vi "TypecastControls.vi"(0 "Controls[]":refnum<vi>[](array[refnum]), 5 "Control Name":string, 9 "Control Path In":string[](array[string]), 11 "error In":errorcluster) -> (4 "Sub Controls[]":refnum<vi>[](array[refnum]), 10 "Control Path Out":string[](array[string]), 15 "error out":errorcluster)   [LabVIEW 2016, in "Drona.lvlib" / "GetControlRef.lvlib"]
doc: "Typecasts the control to its respective class and gives the reference of the controls inside it."
uses:
  GetControlRef.lvlib
  Drona.lvlib
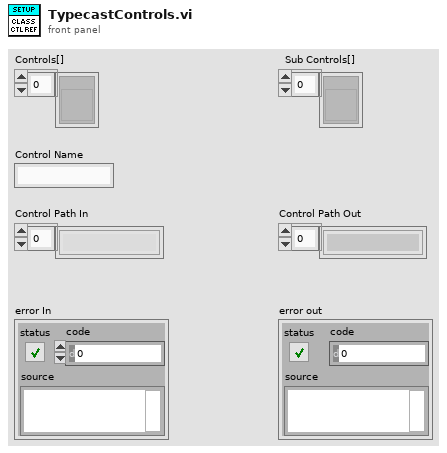
[diagram p1: front panel]
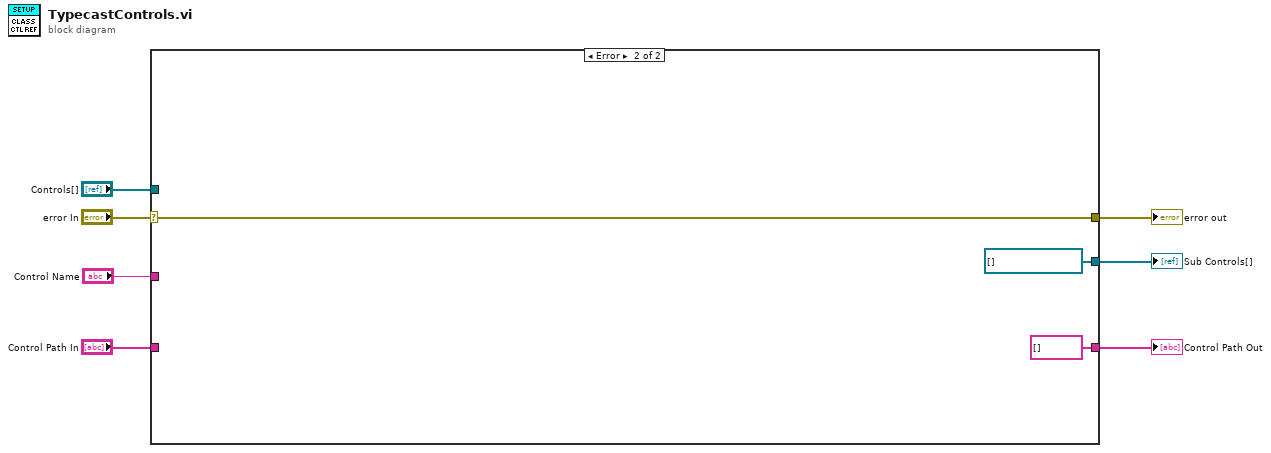
[diagram p0: block diagram]
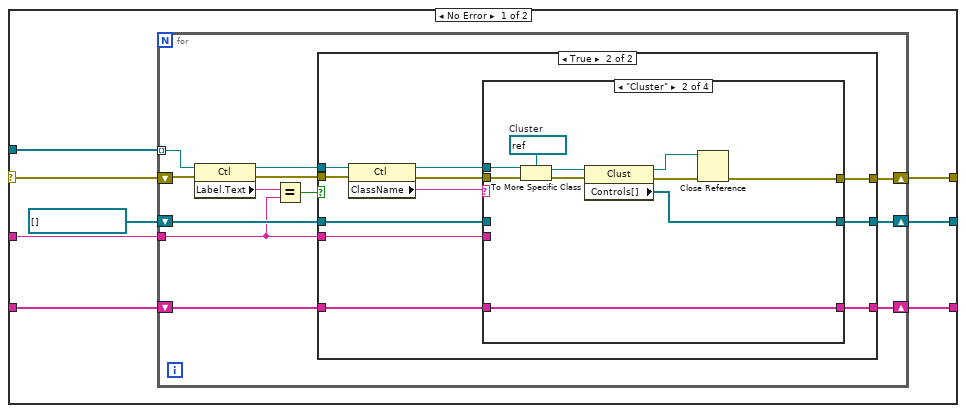
[diagram p2: hidden frame]
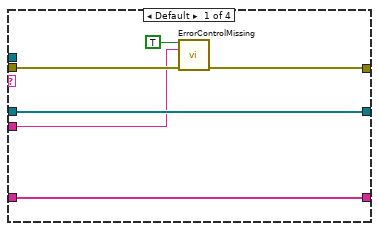
[diagram p4: hidden frame]
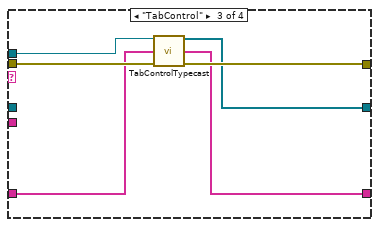
[diagram p5: hidden frame]
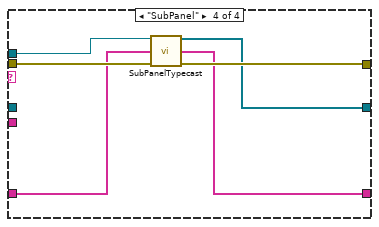
[diagram p6: hidden frame]
diagram:
  n1 = case shown="Error" "error In" {
    selector: "error In" -> [w13 w72]
    tunnel: "Controls[]" -> [w15 _]
    tunnel: "Control Name" -> [w14 _]
    tunnel: [w12 w72] -> w4
    tunnel: [w11 refnum<vi>[] [] ("Controls[]")] -> w3
    tunnel: "Control Path In" -> [w10 _]
    tunnel: [w9 string[] [] ("Control Path In")] -> w1
    frame No Error {
      n2 = for {
        tunnel: w15 -> [w27] mode=indexing
        tunnel: w14 -> [w16]
        shift-right: [w22] -> w11
        shift-left: refnum<vi>[] [] ("Controls[]") -> [w21]
        shift-right: [w20] -> w12
        shift-left: w13 -> [w19]
        shift-right: [w17] -> w9
        shift-left: w10 -> [w18]
        n3 = property class="Ctl"(reference=w27, error in=w19) -> (reference out=w23:refnum<vi>, error out=w24:errorcluster, "Label.Text"=w26:string)
        n4 = Equal?(x=w26, y=w16) -> (x = y?=w25:bool)
        n5 = case shown="True" w25 {
          tunnel: w24 -> [w29 w41]
          tunnel: w23 -> [_ w40]
          tunnel: [w30 w36] -> w22
          tunnel: w21 -> [w30 w34]
          tunnel: [w29 w35] -> w20
          tunnel: w18 -> [w28 w33]
          tunnel: [w28 w32] -> w17
          tunnel: w16 -> [_ w31]
          frame False {
          }
          frame True {
            n6 = property class="Ctl"(reference=w40, error in=w41) -> (reference out=w37:refnum<vi>, error out=w38:errorcluster, "ClassName"=w39:string)
            n7 = case shown="\"Cluster\"" w39 {
              tunnel: w38 -> [w45 w57 w63 w69]
              tunnel: w37 -> [_ w56 w62 w65]
              tunnel: [w47 w52 w58 w64] -> w36
              tunnel: [w44 w50 w60 w68] -> w35
              tunnel: w34 -> [w47 _ _ _]
              tunnel: w33 -> [w46 w48 w61 w67]
              tunnel: [w46 w48 w59 w66] -> w32
              tunnel: w31 -> [w42 _ _ _]
              frame Default {
                n8 = call "ErrorControlMissing.vi"("Create Error?"=TRUE, "Control Name"=w42, "error in"=w45) -> ("error out"=w44:errorcluster)  [unwired: 12 in]
              }
              frame "Cluster" {
                w55 = refnum<vi> refnum  # Cluster
                n9 = To More Specific Class(target class=w55, reference=w56, error in=w57) -> (specific class reference=w54:refnum<vi>, error out=w53:errorcluster)
                n10 = property class="Clust"(reference=w54, error in=w53) -> (reference out=w49:refnum<vi>, error out=w51:errorcluster, "Controls[]"=w52:refnum<vi>[])
                n11 = Close Reference(reference=w49, error in (no error)=w51) -> (error out=w50:errorcluster)
              }
              frame "TabControl" {
                n12 = call "TabControlTypecast.vi"("Ctl Refnum"=w62, "Control Path In"=w61, "Error In"=w63) -> ("Controls[]"=w58:refnum<vi>[], "Control Path Out"=w59:string[], "Error Out"=w60:errorcluster)  [unwired: 10 in]
              }
              frame "SubPanel" {
                n13 = call "SubPanelTypecast.vi"("Ctl Refnum"=w65, "Control Path In"=w67, "Error In"=w69) -> ("Controls[]"=w64:refnum<vi>[], "Control Path Out"=w66:string[], "Error Out"=w68:errorcluster)  [unwired: 10 in]
              }
            }
          }
        }
      }
    }
    frame Error {
    }
  }
  "error out" <- w4
  "Sub Controls[]" <- w3
  "Control Path Out" <- w1
